vi "List_Users_Display.vi"(8 "error in (no error)":errorcluster, 11 "Enum":T1) -> (0 "error out":errorcluster, 3 "Array":string[](array[string]))   [LabVIEW 2021]
uses:
  Control/login_type.ctl
panel:
  out "appended path":path
  out "concatenated string":string
  out "standard output":string
  out "standard error":string
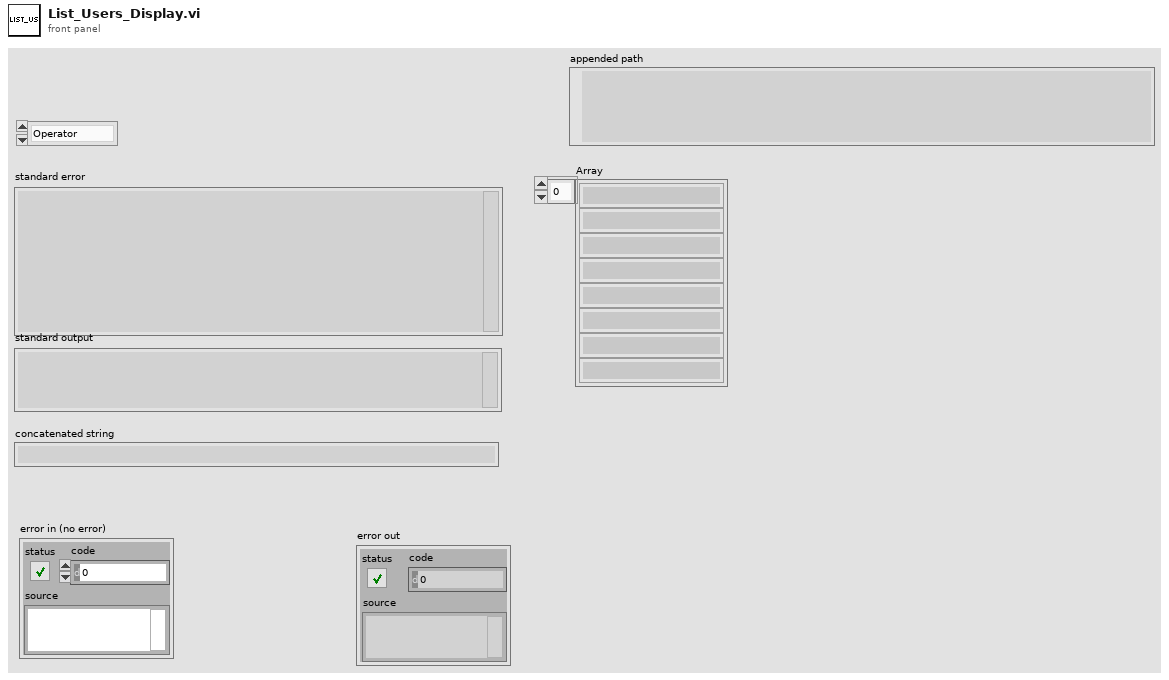
[diagram p1: front panel]
types:
  T1 = typedef "login_type.ctl" = enum16{"Operator", "Admin"}
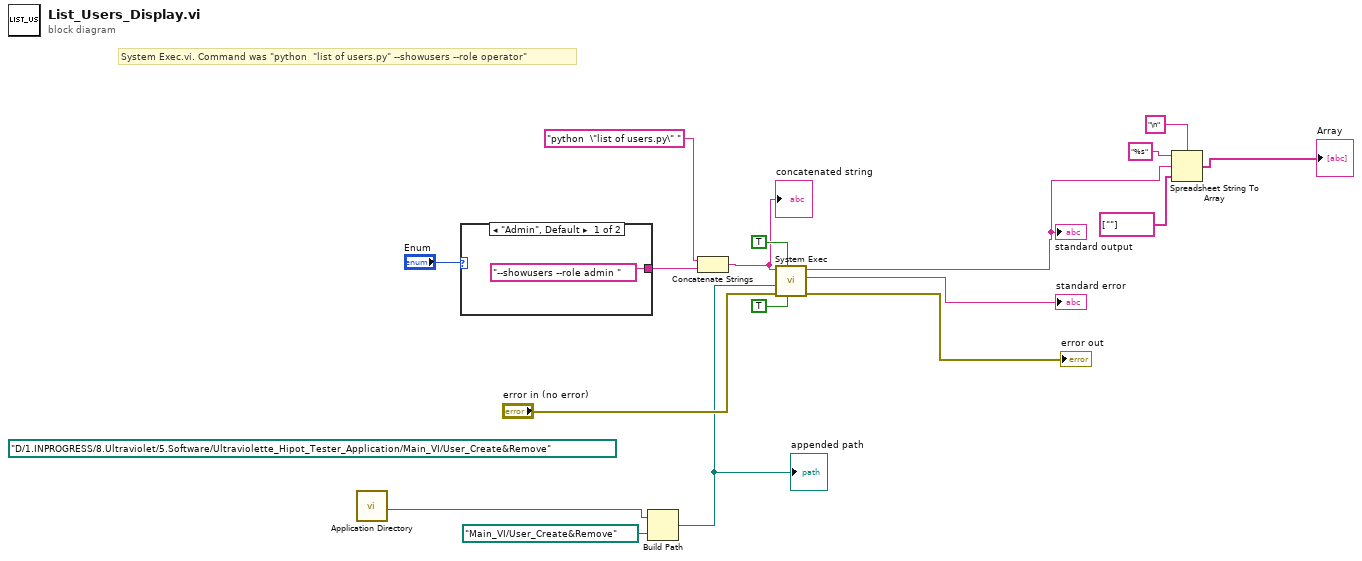
[diagram p0: block diagram]
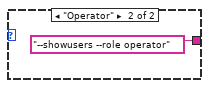
[diagram p2: hidden frame]
diagram:
  (unwired) path "D:/1.INPROGRESS/8.Ultraviolet/5.Software/Ultraviolette_Hipot_Tester_Application/Main_VI/User_Create&Remove" ("working directory")
  # "System Exec.vi. Command was \"python  \"list of users.py\" --showusers --role operator\""
  n1 = call <vilib>:"Application Directory.vi"() -> ("Application Directory"=w2:path)
  n2 = case shown="\"Admin\", Default" "Enum" {
    tunnel: ["--showusers --role admin " ("string") "--showusers --role operator" ("string")] -> w4
    frame "Admin", Default {
    }
    frame "Operator" {
    }
  }
  n3 = Build Path(base path=w2, name or relative path=path "Main_VI/User_Create&Remove") -> (appended path=w1:path)
  "appended path" <- w1
  n4 = Concatenate Strings("python  \"list of users.py\" " ("command line"), w4) -> (w6:string)
  "concatenated string" <- w6
  n5 = call <vilib>:"System Exec.vi"("run minimized? (F)"=TRUE, "wait until completion? (T)"=TRUE, "error in (no error)"="error in (no error)", "working directory"=w1, "command line"=w6) -> ("error out"=→"error out":errorcluster, "standard error"=→"standard error":string, "standard output"=w11:string)  [unwired: 3 in, 1 out]
  "standard output" <- w11
  n6 = Spreadsheet String To Array(delimiter (Tab)="\n", format string="%s", spreadsheet string=w11, array type (2D Dbl)=string[] [""]) -> (array=→"Array":string[])
